vi "Regex Full Probe.vi"(0 "in input string":string, 1 "in ignore case":bool, 2 "in multiline":bool, 5 "in regular expression":string, 7 "in offset":i32, 11 "error in":errorcluster) -> (3 "out matched substrings":string[](array[string]), 4 "out whole match":string, 6 "out before match":string, 8 "out after match":string, 10 "out whole match offset":i32, 15 "error out":errorcluster)   [LabVIEW 2026]
doc: "Probe: every terminal of Match Regular Expression_Execute.vi wired, to map its slots onto the XNode's after Replace."
uses:
  <vilib>/regexp/Match Regular Expression.xnode
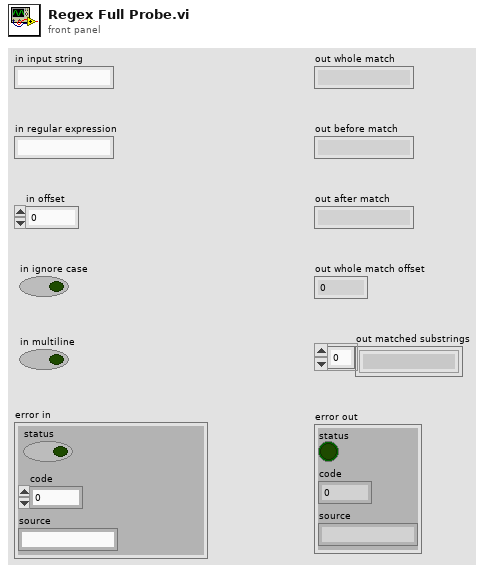
[diagram p1: front panel]
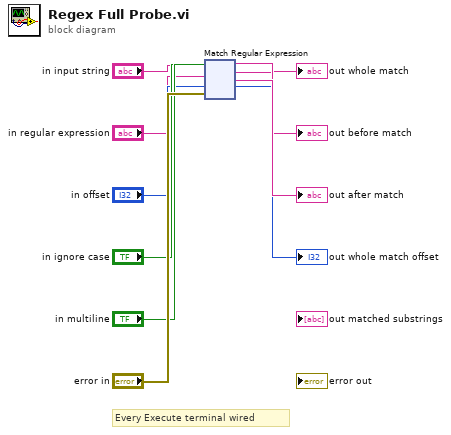
[diagram p0: block diagram]
diagram:
  # "Every Execute terminal wired"
  n1 = xnode "Match Regular Expression"("input string"="in input string", "regular expression"="in regular expression", "offset (0)"="in offset", "error in"="error in", "ignore case? (F)"="in ignore case", "multiline? (F)"="in multiline") -> ("before match"=→"out before match":string, "whole match"=→"out whole match":string, "after match"=→"out after match":string, "offset past match"=→"out whole match offset":i32)  [unwired: 1 out]
